vi "FuncVI-vhConf.vi"(5 "InstanceRef":T2, 9 "arg list":T1[](array[typedef]) {"num" format="%.2f"}) -> (0 "error out":bool, 3 "result":T1 {"num" format="%.2f"})   [LabVIEW 2021]
doc: "::: CalcExpress Toolkit :::\nCopyright (c) 2000-2026 Konstantin Shifershteyn. All rights reserved."
uses:
  cetypes.llb/CalcExpress Function Argument Info.ctl
  cetypes.llb/CalcExpress Instance RefNum.ctl
panel:
  in  "max arg num":i32=7
  in  "min arg num":i32=1
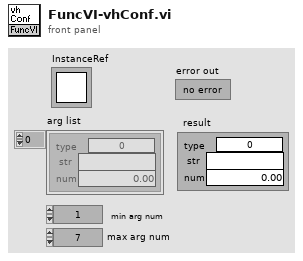
[diagram p1: front panel]
types:
  T1 = typedef "CalcExpress Function Argument Info.ctl" = cluster{"type":u32, "str":string, "num":dbl}
  T2 = typedef "CalcExpress Instance RefNum.ctl" = refnum<k1>
  T3 = enum32{"String", "DBL Number", "identifier", "1D Array of DBL", "2D Array of DBL", "CDB Number", "1D Array of CDB", "2D Array of CDB", "1D Array of String", "2D Array of String", "Unknown data type"}
  T4 = cluster{"index":i32, "data type":enum32{"String", "DBL Number", "identifier", "1D Array of DBL", "2D Array of DBL", "CDB Number", "1D Array of CDB", "2D Array of CDB", "1D Array of String", "2D Array of String", "Unknown data type"}, "default num":dbl, "default str":string}[]
  T5 = enum32{"nop", "create", "destroy", "reset", "get info", "config", "create_wrid"}
  T6 = cluster{"num list[0]":dbl, "num list[1]":dbl, "num list[2]":dbl, "num list[3]":dbl, "num list[4]":dbl, "num list[5]":dbl, "num list[6]":dbl}
  T7 = cluster{u32, "num list[4]":dbl, "num list[5]":dbl, "num list[6]":dbl}
  T8 = typedef "VarMan Variable Context Handle.ctl" = i32
  T9 = cluster{"data type":enum32{"String", "DBL Number", "identifier", "1D Array of DBL", "2D Array of DBL", "CDB Number", "1D Array of CDB", "2D Array of CDB", "1D Array of String", "2D Array of String", "Unknown data type"}, string, dbl}
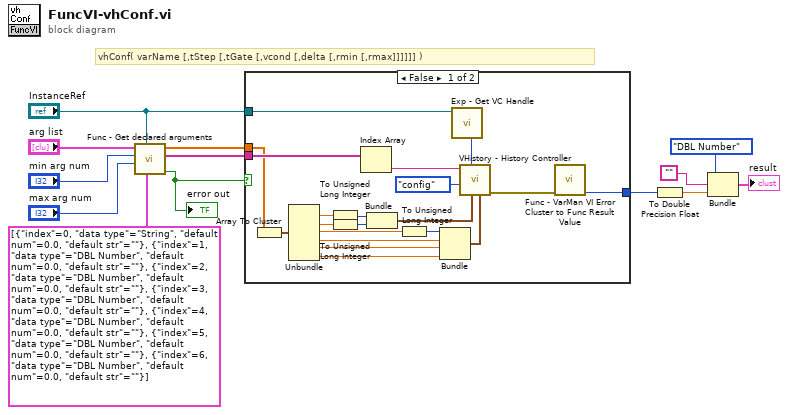
[diagram p0: block diagram]
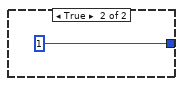
[diagram p2: hidden frame]
diagram:
  # "vhConf( varName [,tStep [,tGate [,vcond [,delta [,rmin [,rmax]]]]]] )"
  n1 = call "Func - Get declared arguments.vi"("arg descriptors"=T4 [{"index"=0, "data type"=enum."String", "default num"=0.0, "default str"=""}, {"index"=1, "data type"=enum."DBL Number", "default num"=0.0, "default str"=""}, {"index"=2, "data type"=enum."DBL Number", "default num"=0.0, "default str"=""}, {"index"=3, "data type"=enum."DBL Number", "default num"=0.0, "default str"=""}, {"index"=4, "data type"=enum."DBL Number", "default num"=0.0, "default str"=""}, {"index"=5, "data type"=enum."DBL Number", "default num"=0.0, "default str"=""}, {"index"=6, "data type"=enum."DBL Number", "default num"=0.0, "default str"=""}], "InstanceRef"="InstanceRef", "max arg num"="max arg num", "min arg num"="min arg num", "arg list"="arg list") -> ("error out"=w12:bool, "str list"=w8:string[], "num list"=w1:dbl[])  [unwired: 3 in, 1 out]
  "error out" <- w12
  n2 = case shown="False" w12 {
    tunnel: w1 -> [w19 _]
    tunnel: w8 -> [w33 _]
    tunnel: [w15 1 ("code")] -> w7
    tunnel: "InstanceRef" -> [w31 _]
    frame False {
      n3 = Array To Cluster(array=w19) -> (cluster=w20:T6)
      n4 = Unbundle(w20) -> ("num list[1]"=w17:dbl, "num list[2]"=w18:dbl, "num list[3]"=w21:dbl, "num list[4]"=w24:dbl, "num list[5]"=w25:dbl, "num list[6]"=w26:dbl)  [unwired: 1 out]
      n5 = To Unsigned Long Integer(number=w17) -> (unsigned 32bit integer=w29:u32)
      n6 = To Unsigned Long Integer(number=w18) -> (unsigned 32bit integer=w28:u32)
      n7 = Index Array(array=w33) -> (element=w32:string)  [unwired: 1 in]
      n8 = Bundle(w29, w28) -> (w27:cluster{u32, u32})  [unwired: 1 in]
      n9 = To Unsigned Long Integer(number=w21) -> (unsigned 32bit integer=w22:u32)
      n10 = Bundle(w22, "num list[4]"=w24, "num list[5]"=w25, "num list[6]"=w26) -> (w23:T7)  [unwired: 1 in]
      n11 = call "Exp - Get VC Handle.vi"("InstanceRef"=w31) -> ("VC Handle"=w30:T8)  [unwired: 5 in, 3 out]
      n12 = call "VHistory - History Controller.vi"("value condition"=w23, "time conditions"=w27, "VC Handle"=w30, "cmd (nop:default)"=T5."config", "name_spec"=w32) -> ("error out"=w16:errorcluster)  [unwired: 3 in, 3 out]
      n13 = call "Func - VarMan VI Error Cluster to Func Result Value.vi"("VarMan VI error in"=w16) -> ("CE Function Result Value"=w15:i32)  [unwired: 10 in]
    }
    frame True {
    }
  }
  n14 = To Double Precision Float(number=w7) -> (double precision float=w6:dbl)
  n15 = Bundle("data type"=T3."DBL Number", "", w6) -> (→"result":T9)  [unwired: 1 in]
